vi "Memory Data Mode Enabled.vi"(8 "error in (no error)":errorcluster caption="错误输入（无错误）") -> (0 "error out":errorcluster caption="错误输出", 3 "function return":bool)   [LabVIEW 2017, in "smncsftmt.lvlib"]
doc: "__declspec(dllexport) bool MemoryDataModeEnabled();"
uses:
  smncsftmt.lvlib
  smncsftmt.dll
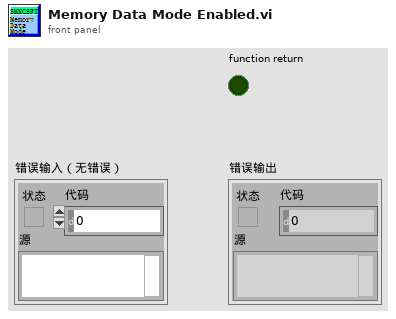
[diagram p1: front panel]
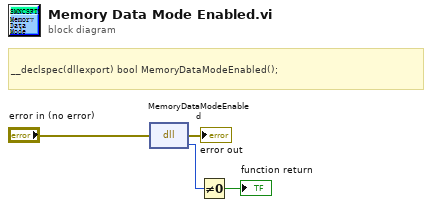
[diagram p0: block diagram]
diagram:
  # "__declspec(dllexport) bool MemoryDataModeEnabled();"
  n1 = dll-call lib="PTH2oabs CUsersaDesktop\nLABVIEW范例National InstrumentsLabVIEW 2017user.lib\tsmncsftmtsmncsftmt.*" fn="MemoryDataModeEnabled"(error in="error in (no error)") -> (error out=→"error out":errorcluster, w3:u8)  [unwired: 2 in, 1 out]
  n2 = Not Equal To 0?(x=w3) -> (x != 0?=→"function return":bool)
